vi "Read Binary File.vi"(11 "路径":path=path "C:/Users/P53/Desktop/t1.dat") -> (0 "错误输出":errorcluster, 3 "数据系列":T1[](array[typedef]))   [LabVIEW 2020, in "Data Viewer.lvlib" / "Data Viewer.lvclass"]
uses:
  Data Viewer.lvclass
  Data Serie--cluster.ctl
  Data Viewer.lvlib
panel:
  in  "排列方式":enum16{"按列排列", "按行排列"}(ring)=enum."按行排列"
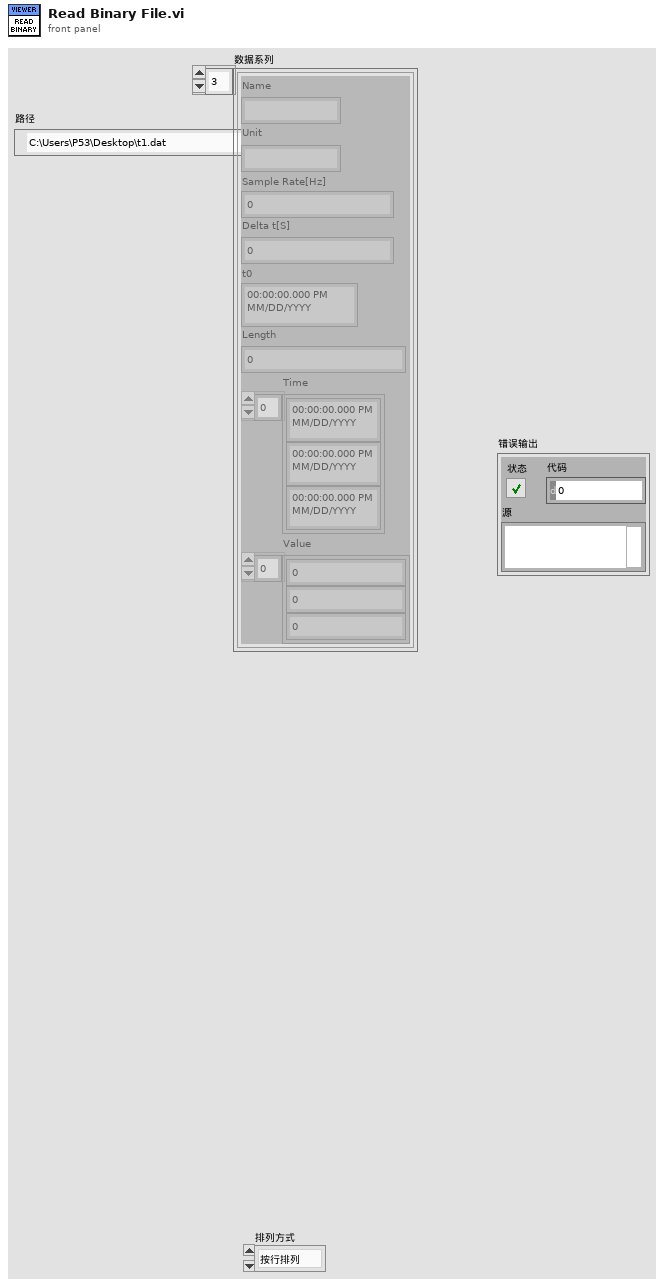
[diagram p1: front panel]
types:
  T1 = typedef "Data Viewer.lvlib/Data Serie--cluster.ctl" = cluster{"Name":string, "Unit":string, "Sample Rate[Hz]":dbl, "Delta t[S]":dbl, "t0":timestamp, "Length":i32, "Time":timestamp[], "Value":dbl[]}
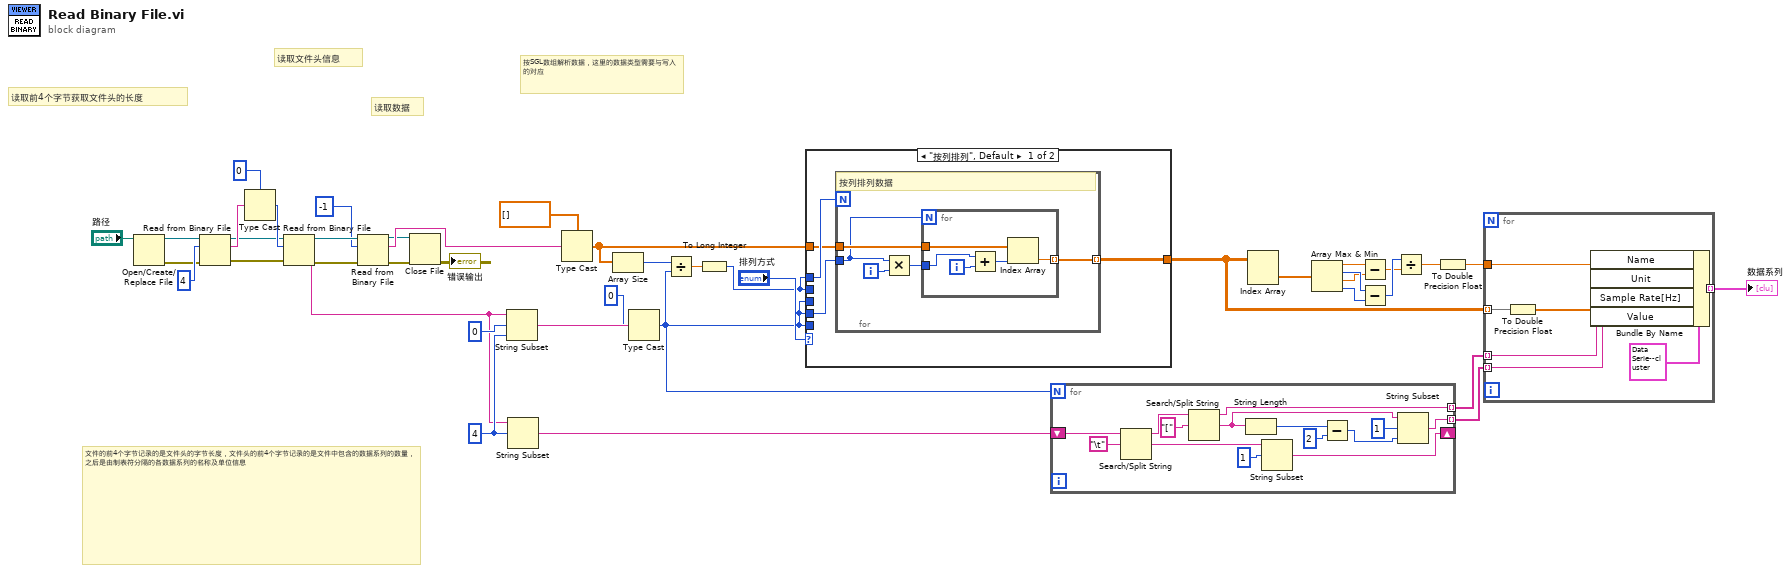
[diagram p0: block diagram]
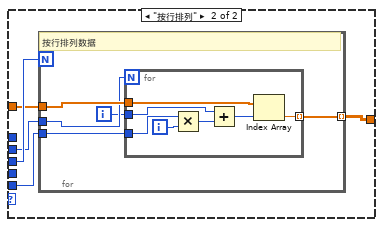
[diagram p2: hidden frame]
diagram:
  w31 = 4 ("长度（剩余）")
  # "文件的前4个字节记录的是文件头的字节长度，文件头的前4个字节记录的是文件中包含的数据系列的数量，之后是由制表符分隔的各数据系列的名称及单位信息"
  # "按SGL数组解析数据，这里的数据类型需要与写入的对应"
  # "读取数据"
  # "读取文件头信息"
  # "读取前4个字节获取文件头的长度"
  n1 = Open/Create/Replace File(file path (use dialog)="路径") -> (refnum out=w41:refnum<file>, error out=w6:errorcluster)  [unwired: 5 in, 1 out]
  n2 = Read from Binary File(8:w6, 10:4 ("总数(1)"), 11:w41) -> (0:w5:errorcluster, 2:w39:string, 3:w36:refnum<file>)  [unwired: 3 in, 1 out]
  n3 = Type Cast(type=0, x=w39) -> (*(type *) &x=w37:i32)
  n4 = Read from Binary File(8:w5, 10:w37, 11:w36) -> (0:w4:errorcluster, 2:w28:string, 3:w35:refnum<file>)  [unwired: 3 in, 1 out]
  n5 = Read from Binary File(8:w4, 10:-1 ("总数(1)"), 11:w35) -> (0:w3:errorcluster, 2:w33:string, 3:w2:refnum<file>)  [unwired: 3 in, 1 out]
  n6 = Close File(refnum=w2, error in=w3) -> (error out=→"错误输出":errorcluster)  [unwired: 1 out]
  n7 = String Subset(string=w28, offset (0)=0 ("偏移量(0)"), length (rest)=w31) -> (substring=w30:string)
  n8 = String Subset(string=w28, offset (0)=w31) -> (substring=w20:string)  [unwired: 1 in]
  n9 = Type Cast(type=sgl[] [], x=w33) -> (*(type *) &x=w23:sgl[])
  n10 = Array Size(array=w23) -> (size(s)=w26:i32)
  n11 = Type Cast(type=0, x=w30) -> (*(type *) &x=w21:i32)
  n12 = Divide(x=w26, y=w21) -> (x/y=w25:dbl)
  n13 = To Long Integer(number=w25) -> (32bit integer=w22:i32)
  n14 = case shown="\"按列排列\", Default" "排列方式" {
    tunnel: [w46 w57] -> w11
    tunnel: w22 -> [w45 _]
    tunnel: w21 -> [w44 _]
    tunnel: w21 -> [_ w61]
    tunnel: w23 -> [w43 w60]
    tunnel: w22 -> [_ w59]
    tunnel: w21 -> [_ w58]
    frame "按列排列", Default {
      n15 = for {
        N: w45 -> [_]
        tunnel: w43 -> [w51]
        tunnel: w44 -> [w47]
        tunnel: [w48] -> w46 mode=indexing
        i -> [w50]
        # "按列排列数据"
        n16 = Multiply(x=w47, y=w50) -> (x*y=w49:i32)
        n17 = for {
          N: w47 -> [_]
          tunnel: w51 -> [w56]
          tunnel: w49 -> [w53]
          tunnel: [w52] -> w48 mode=indexing
          i -> [w55]
          n18 = Add(x=w53, y=w55) -> (x+y=w54:i32)
          n19 = Index Array(array=w56, index=w54) -> (element=w52:sgl)
        }
      }
    }
    frame "按行排列" {
      n20 = for {
        N: w61 -> [_]
        tunnel: w60 -> [w66]
        tunnel: w59 -> [w65]
        tunnel: [w63] -> w57 mode=indexing
        tunnel: w58 -> [w62]
        i -> [w64]
        # "按行排列数据"
        n21 = for {
          N: w65 -> [_]
          tunnel: w66 -> [w73]
          tunnel: w64 -> [w70]
          tunnel: [w68] -> w63 mode=indexing
          tunnel: w62 -> [w67]
          i -> [w72]
          n22 = Multiply(x=w67, y=w72) -> (x*y=w71:i32)
          n23 = Add(x=w70, y=w71) -> (x+y=w69:i32)
          n24 = Index Array(array=w73, index=w69) -> (element=w68:sgl)
        }
      }
    }
  }
  n25 = for {
    N: w21 -> [_]
    tunnel: [w79] -> w19 mode=indexing
    tunnel: [w78] -> w18 mode=indexing
    shift-right: [w75] -> _
    shift-left: w20 -> [w74]
    n26 = Search/Split String(string=w74, search string/char (-)="\t") -> (substring before match=w80:string, match + rest of string=w77:string)  [unwired: 1 in, 1 out]
    n27 = Search/Split String(string=w80, search string/char (-)="[" ("搜索字符串/字符(-)")) -> (substring before match=w79:string, match + rest of string=w84:string)  [unwired: 1 in, 1 out]
    n28 = String Length(string=w84) -> (length=w82:i32)
    n29 = String Subset(string=w77, offset (0)=1 ("偏移量(0)")) -> (substring=w75:string)  [unwired: 1 in]
    n30 = Subtract(x=w82, y=2) -> (x-y=w83:i32)
    n31 = String Subset(string=w84, offset (0)=1 ("偏移量(0)"), length (rest)=w83) -> (substring=w78:string)
  }
  n32 = Index Array(array=w11) -> (element=w12:sgl[])  [unwired: 2 in]
  n33 = Array Max & Min(array=w12) -> (max value=w13:sgl, max index (indices)=w15:i32, min value=w14:sgl, min index (indices)=w9:i32)
  n34 = Subtract(x=w13, y=w14) -> (x-y=w16:sgl)
  n35 = Subtract(x=w15, y=w9) -> (x-y=w17:i32)
  n36 = Divide(x=w17, y=w16) -> (x/y=w10:sgl)
  n37 = To Double Precision Float(number=w10) -> (double precision float=w8:dbl)
  n38 = for {
    tunnel: w19 -> [w94] mode=indexing
    tunnel: w18 -> [w93] mode=indexing
    tunnel: w11 -> [w92] mode=indexing
    tunnel: w8 -> [w90]
    tunnel: [w89] -> w7 mode=indexing
    n39 = To Double Precision Float(number=w92) -> (double precision float=w91:dbl[])
    n40 = Bundle By Name(cluster=T1 {"Name"="", "Unit"="", "Sample Rate[Hz]"=0.0, "Delta t[S]"=0.0, "t0"=timestamp(0 s since 1904-01-01), "Length"=0, "Time"=[], "Value"=[]} ("Data Serie"), "Name"=w94, "Unit"=w93, "Sample Rate[Hz]"=w90, "Value"=w91) -> (w89:T1)
  }
  "数据系列" <- w7
